vi "optical_camera_images.vi"() -> ()   [LabVIEW 2025]
panel:
  in  "Capture\nStart/Stop":bool
  in  "Stop (F)":bool
  in  "Acquisition Control:\nExposure Time [100, 3E7]":dbl=999.0 caption="Acquisition Control::Exposure Time" min=100.0 max=29999995.0
  in  "Analog Control:\nGain [0, 27]":dbl caption="Analog Control::Gain" min=0.0 max=27.045663671679687
  in  "Analog Control:\nBlack Level [-5, 10]":dbl caption="Analog Control::Black Level" min=-5.0000011920928955 max=10.000002384185791
  in  "Analog Control:\nGamma [0.25, 4.00]":dbl=0.800048828125 caption="Analog Control::Gamma" min=0.25 max=4.0 step=0.05
  out "Optical camera":T1(plugin-control)
  in  "optical capture interval (s)":dbl
  in  "File Path":string="C:\\Digambar\\Metal_thin_wall\\Optical_images\\Optical_images"
  out "File Name Out":string
  # "Destination for Optical Images:"
  # "change folder names each time you run,\nso it saves data sets in dedicated folders:\nfolder1\nfolder2\nfolder3\netc..."
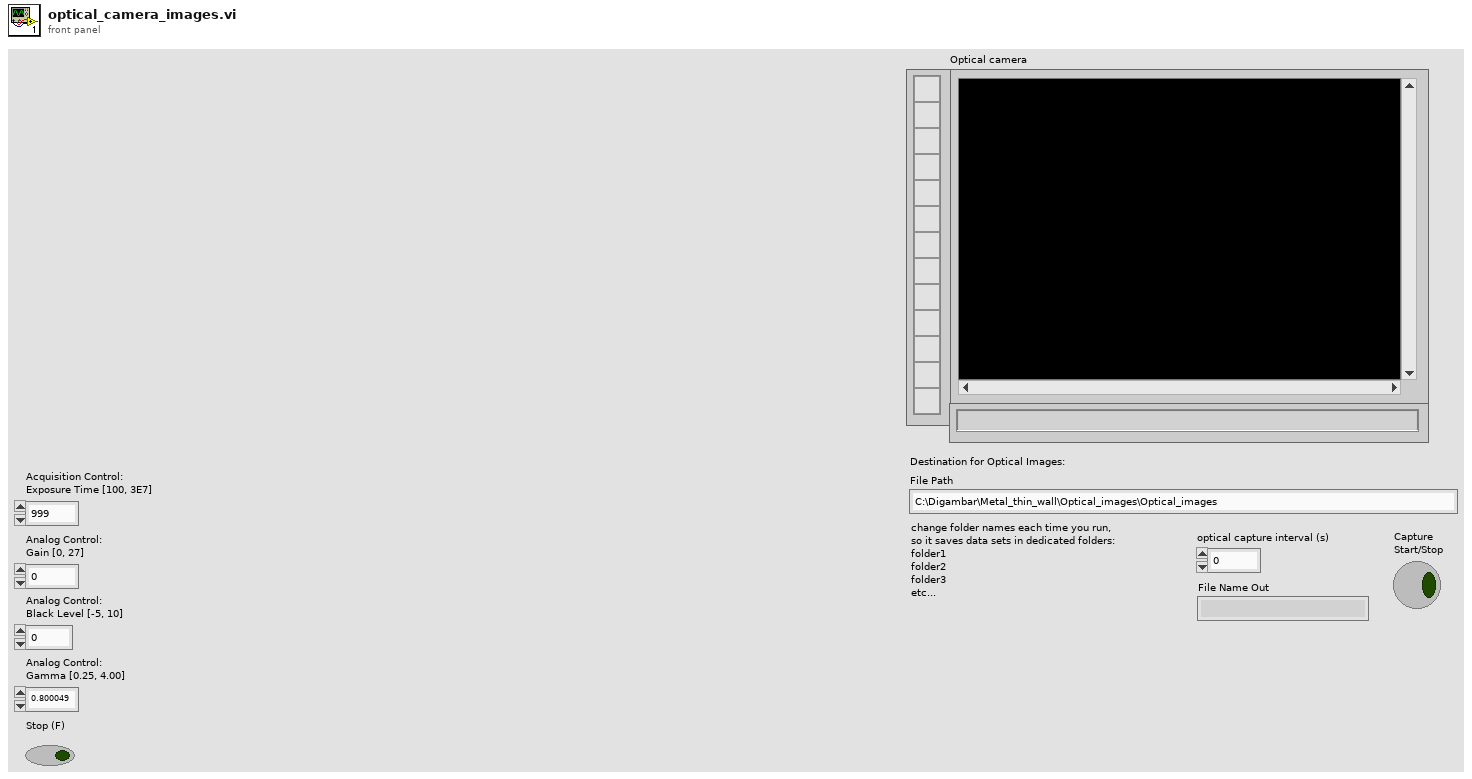
[diagram p1: front panel]
types:
  T1 = typedef "IMAQ Image.ctl" = refnum<image>
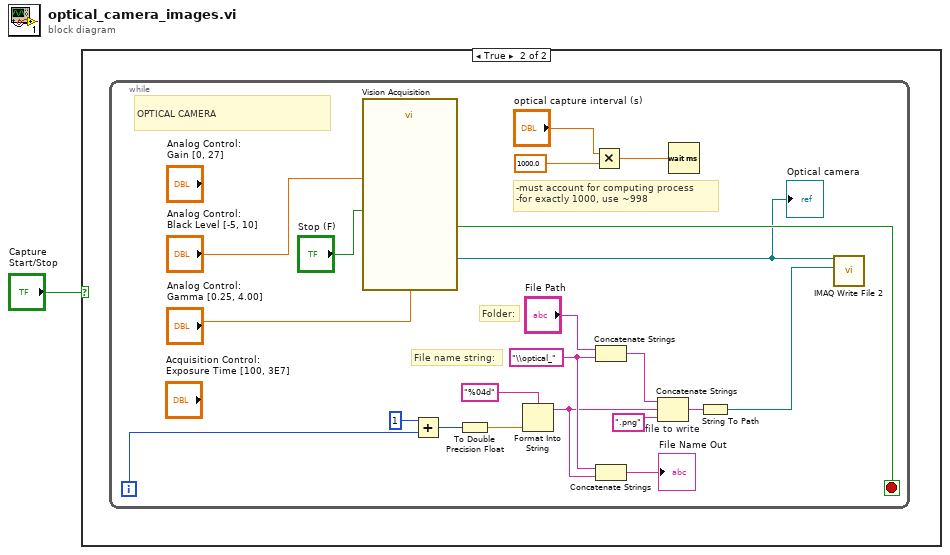
[diagram p0: block diagram]
diagram:
  n1 = case shown="True" "Capture\nStart/Stop" {
    frame False {
    }
    frame True {
      n2 = while {
        i -> [w3]
        stop <- w21 stop-if-true
        w9 = "\\optical_" ("string")
        # "-must account for computing process\n-for exactly 1000, use ~998"
        # "OPTICAL CAMERA"
        # "Folder:"
        # "File name string:"
        n3 = call "Vision Acquisition"("Analog Control::Black Level"="Analog Control:\nBlack Level [-5, 10]", "Analog Control::Gamma"="Analog Control:\nGamma [0.25, 4.00]", "Stop (F)"="Stop (F)") -> ("Image Out"=w20:T1, "Stopped"=w21:bool)  [unwired: 22 in, 1 out]
        "Optical camera" <- w20
        n4 = Add(x=1, y=w3) -> (x+y=w2:i32)
        n5 = To Double Precision Float(number=w2) -> (double precision float=w5:dbl)
        n6 = Format Into String(format string="%04d" ("time format string (%c)"), w5) -> (resulting string=w7:string)  [unwired: 2 in, 1 out]
        n7 = Multiply(x="optical capture interval (s)", y=1000.0) -> (x*y=w15:dbl)
        n8 = Concatenate Strings("File Path", w9) -> (w10:string)
        n9 = Concatenate Strings(w9, w7) -> (→"File Name Out":string)
        n10 = Concatenate Strings "file to write"(w10, w7, ".png" ("string")) -> (w17:string)
        n11 = Wait (ms)(milliseconds to wait=w15) -> ()  [unwired: 1 out]
        n12 = String To Path(string=w17) -> (path=w13:path)
        n13 = call-poly "IMAQ Write File 2"("File Path"=w13, "Image"=w20) -> ()  [unwired: 8 in, 2 out]
      }
    }
  }
